vi "Server.vi"() -> ()   [LabVIEW 2014]
uses:
  <vilib>/OPCUA/NI OPC UA Server.lvlib
  OPCUA XML/OPCUA XML(dev).lvlib
panel:
  out "xml path":path
  out "trusted client certfications":path[](array[path])
  out "Parse Errors":string
  out "ready":bool
  out "server endpoint URL":string
  in  "show structure":bool
  out "error out":errorcluster
  in  "stop":bool
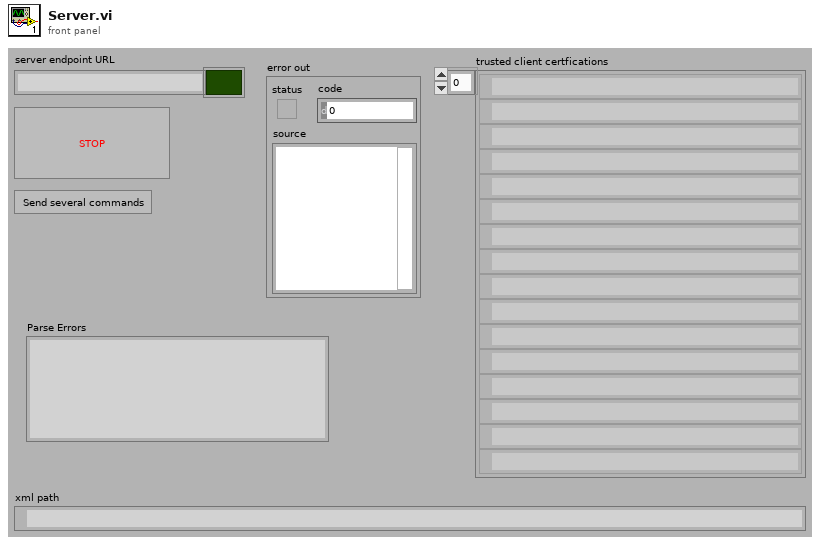
[diagram p1: front panel]
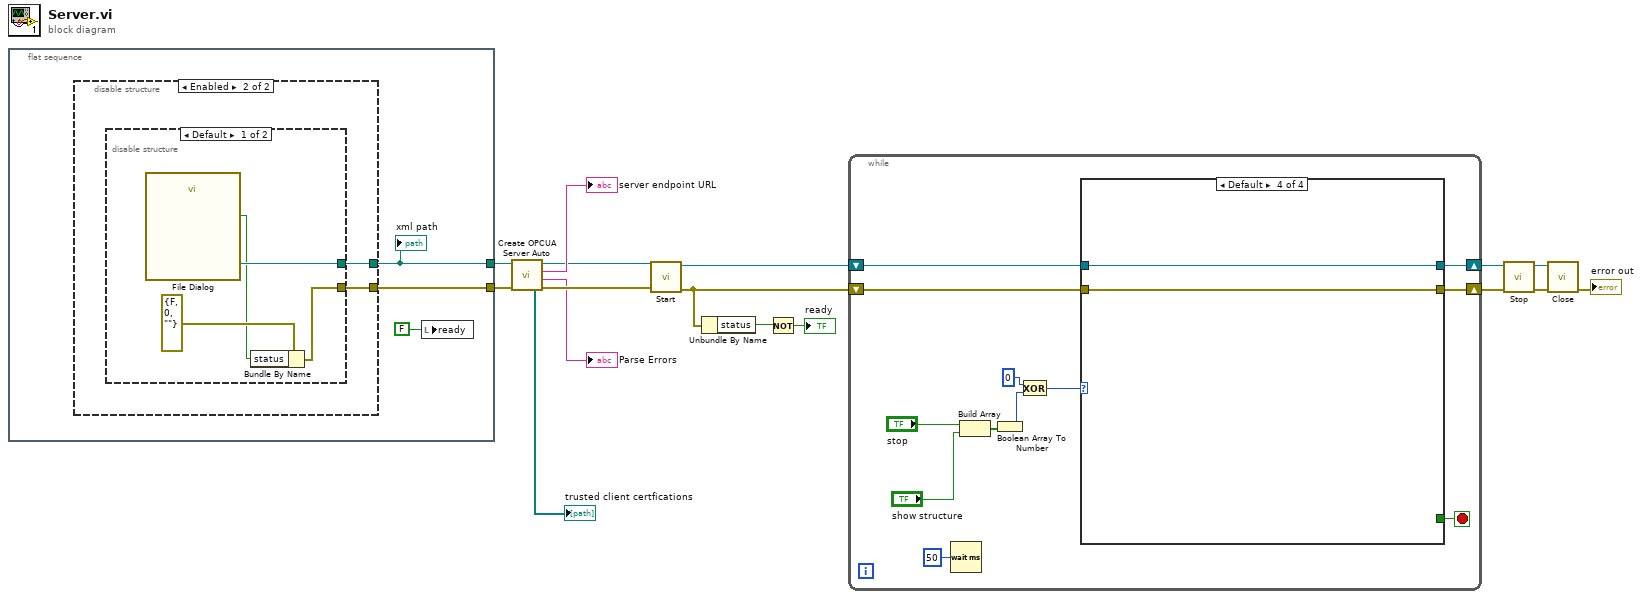
[diagram p0: block diagram]
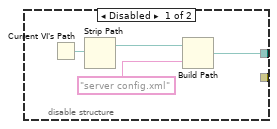
[diagram p2: hidden frame]
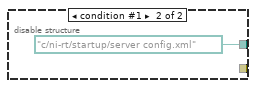
[diagram p3: hidden frame]
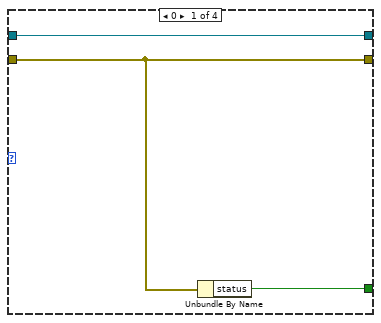
[diagram p4: hidden frame]
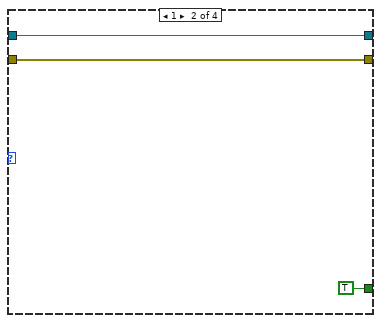
[diagram p5: hidden frame]
diagram:
  n1 = flat-sequence {
    tunnel: [w18] -> w2
    tunnel: [w17] -> w1
    frame #0 {
      n2 = disable-structure shown="Enabled" {
        disable-tunnel: [w20 w25] -> w18
        disable-tunnel: [_ w24] -> w17
        frame Disabled {
          n3 = Current VI's Path() -> (path=w23:path)
          n4 = Strip Path(path=w23) -> (stripped path=w22:path)  [unwired: 1 out]
          n5 = Build Path(base path=w22, name or relative path="server config.xml") -> (appended path=w20:path)
        }
        frame Enabled {
          n6 = disable-structure shown="Default" {
            disable-tunnel: [w29 path "c:/ni-rt/startup/server config.xml" ("selected path")] -> w25
            disable-tunnel: [w26 _] -> w24
            frame condition #0 (active) {
              n7 = call "File Dialog"() -> ("selected path"=w29:path, "cancelled"=w27:bool)  [unwired: 12 in, 2 out]
              n8 = Bundle By Name(cluster=errorcluster {"status"=FALSE, "code"=0, "source"=""} ("error constant"), "status"=w27) -> (w26:errorcluster)
            }
            frame condition #1 {
            }
          }
        }
      }
      "xml path" <- w18
      n9 = local write "ready"(FALSE) -> ()
    }
  }
  n10 = call "Create OPCUA Server Auto.vi"("Error In"=w1, "XML config File Path"=w2) -> ("Error Out"=w5:errorcluster, "Parse Errors"=→"Parse Errors":string, "server endpoint URL"=→"server endpoint URL":string, "OPC UA server refnum out"=w6:refnum<k21>, "trusted client certfications"=→"trusted client certfications":path[])  [unwired: 5 in]
  n11 = call <vilib>:"Start.vi"("error in (no error)"=w5, "OPC UA server refnum in"=w6) -> ("error out"=w9:errorcluster, "OPC UA server refnum out"=w16:refnum<k21>)  [unwired: 8 in]
  n12 = Unbundle By Name(w9) -> ("status"=w8:bool)
  n13 = Not(x=w8) -> (.not. x?=→"ready":bool)
  n14 = while {
    shift-right: [w36] -> w13
    shift-left: w16 -> [w35]
    shift-right: [w33] -> w11
    shift-left: w9 -> [w34]
    stop <- w32 stop-if-true
    n15 = Wait (ms)(milliseconds to wait=u32 50) -> ()  [unwired: 1 out]
    n16 = Build Array("stop", "show structure") -> (w39:bool[])
    n17 = Boolean Array To Number(Boolean array=w39) -> (number=w31:u32)
    n18 = Exclusive Or(1:w31, 2:u32 0) -> (0:w37:u32)
    n19 = case shown="Default" w37 {
      tunnel: [w45 w48 w50 w52] -> w36
      tunnel: w35 -> [w45 w48 w50 w52]
      tunnel: w34 -> [w43 w47 w49 w51]
      tunnel: [w43 w47 w49 w51] -> w33
      tunnel: [w44 TRUE _ _] -> w32
      frame 0 {
        n20 = Unbundle By Name(w43) -> ("status"=w44:bool)
      }
      frame 1 {
      }
      frame 2 {
      }
      frame Default {
      }
    }
  }
  n21 = call <vilib>:"Stop.vi"("error in (no error)"=w11, "OPC UA server refnum in"=w13) -> ("error out"=w10:errorcluster, "OPC UA server refnum out"=w12:refnum<k21>)  [unwired: 8 in]
  n22 = call <vilib>:"Close.vi"("error in (no error)"=w10, "OPC UA server refnum in"=w12) -> ("error out"=→"error out":errorcluster)  [unwired: 9 in]
